vi "SA set Marker OFF.vi"(8 "error in (no error)":errorcluster caption="에러 입력(에러 없음)", 9 "On?":bool, 10 "Marker Index":i32, 11 "Instrument Manager 입력":refnum<class "Instrument Manager.lvclass">) -> (0 "error out":errorcluster caption="에러 출력", 3 "Instrument Manager 출력":refnum<class "Instrument Manager.lvclass">)   [LabVIEW 2023, in "Instrument Manager.lvclass"]
uses:
  Instrument Manager.lvclass
  Module/Spectrum Analyzer/Class/FSV-40N/FSV-40N.lvclass
  Instrument Manager.lvclass/Instrument Manager.ctl
  Module/Spectrum Analyzer/Class/FSV-40N/FSV-40N.lvclass/FSV-40N.ctl
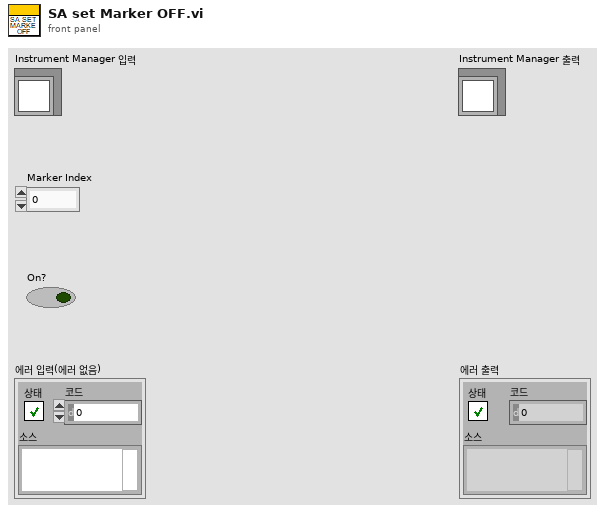
[diagram p1: front panel]
types:
  T1 = cluster{"Anritsu Call Box":refnum<class "Anritsu Call Box.lvclass">, "Spectrum Analyzer":refnum<class "Interface_Spectrum.lvclass">, "RF Switch Box":refnum<class "RF Filter Box.lvclass">, "Turn Table":refnum<class "Interface - Turn Table.lvclass">, "Mast":refnum<class "Interface - Mast.lvclass">, "3D Controller":refnum<class "Interface_3D Controller.lvclass">}
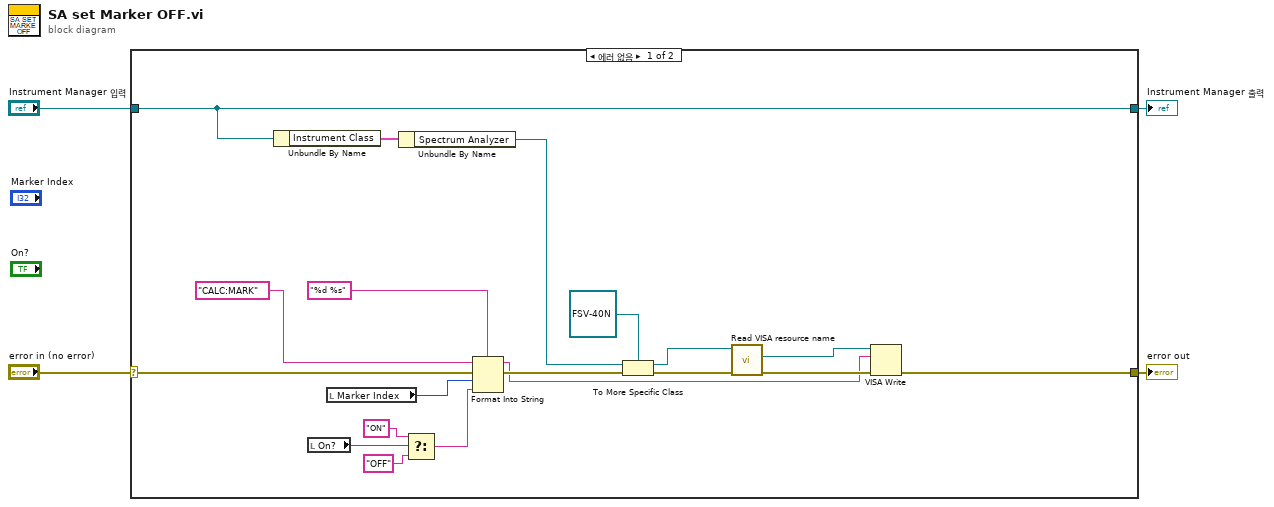
[diagram p0: block diagram]
diagram:
  n1 = case shown="에러 없음" "error in (no error)" {
    selector: "error in (no error)" -> [w19 w25]
    tunnel: [w10 w25] -> w3
    tunnel: [w23 w24] -> w1
    tunnel: "Instrument Manager 입력" -> [w23 w24]
    frame No Error {
      n2 = Unbundle By Name(w23) -> ("Instrument Class"=w22:T1)
      n3 = local read "On?"() -> (w8:bool)
      n4 = local read "Marker Index"() -> (w9:i32)
      n5 = Unbundle By Name(w22) -> ("Spectrum Analyzer"=w18:refnum<class "Interface_Spectrum.lvclass">)
      n6 = Select(t="ON" ("format string"), s=w8, f="OFF" ("format string")) -> (s? t:f=w5:string)
      n7 = Format Into String(format string="%d %s", initial string="CALC:MARK", error in=w19, w9, w5) -> (resulting string=w11:string, error out=w17:errorcluster)
      n8 = To More Specific Class(target class=refnum<class "FSV-40N.lvclass"> refnum ("Spectrum Analyzer.lvlib:FSV-40N.lvclass"), reference=w18, error in=w17) -> (specific class reference=w14:refnum<class "FSV-40N.lvclass">, error out=w15:errorcluster)
      n9 = call "Read VISA resource name.vi"("error in (no error)"=w15, "FSV-40N in"=w14) -> ("error out"=w13:errorcluster, "VISA resource name"=w12:refnum<visa-resource-name>)  [unwired: 7 in, 1 out]
      n10 = VISA Write(VISA resource name=w12, write buffer=w11, error in (no error)=w13) -> (error out=w10:errorcluster)  [unwired: 2 out]
    }
    frame Error {
    }
  }
  "error out" <- w3
  "Instrument Manager 출력" <- w1
